vi "XOR.vi"() -> ()   [LabVIEW 2016]
panel:
  in  "Boolean 4":bool
  in  "Boolean 3":bool
  in  "Boolean 2":bool
  in  "Boolean":bool
  out "GATE RES":bool
  out "CASE RES":bool
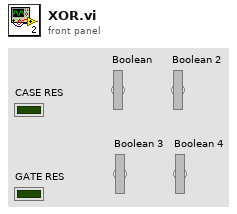
[diagram p1: front panel]
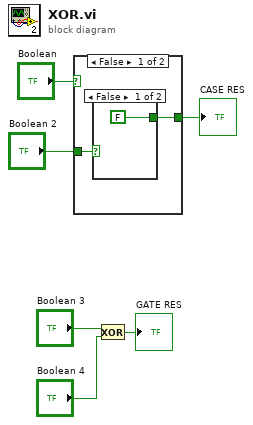
[diagram p0: block diagram]
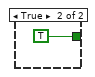
[diagram p2: hidden frame]
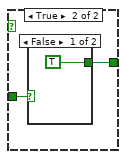
[diagram p3: hidden frame]
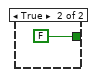
[diagram p4: hidden frame]
diagram:
  n1 = case shown="False" "Boolean" {
    tunnel: [w7 w12] -> w3
    tunnel: "Boolean 2" -> [w8 w11]
    frame False {
      n2 = case shown="False" w8 {
        tunnel: [FALSE TRUE] -> w7
        frame False {
        }
        frame True {
        }
      }
    }
    frame True {
      n3 = case shown="False" w11 {
        tunnel: [TRUE FALSE] -> w12
        frame False {
        }
        frame True {
        }
      }
    }
  }
  "CASE RES" <- w3
  n4 = Exclusive Or(1:"Boolean 4", 2:"Boolean 3") -> (0:→"GATE RES":bool)
